vi "get all the images so i dont have to.vi"() -> ()   [LabVIEW 2021]
panel:
  out "filenames":string[](array[string])
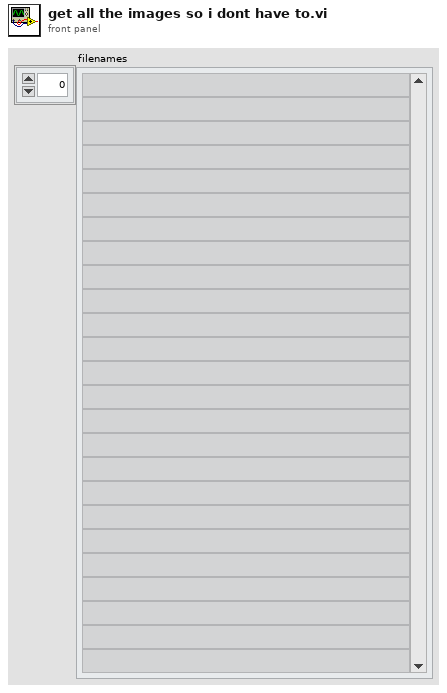
[diagram p1: front panel]
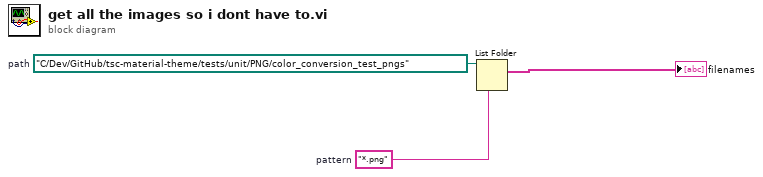
[diagram p0: block diagram]
diagram:
  w2 = path "C:/Dev/GitHub/tsc-material-theme/tests/unit/PNG/color_conversion_test_pngs"  # path
  w3 = "*.png"  # pattern
  n1 = List Folder(path=w2, pattern=w3) -> (filenames=→"filenames":string[])  [unwired: 2 in, 3 out]
